vi "VIH - VI Doc Editor - Dialog - Apply Changes.vi"(7 "Title":string, 11 "msg in":string) -> (0 "action":T1(ring))   [LabVIEW 2014]
doc: "::: VI Helpeks :::\nCopyright (c) 2000-2026 Konstantin Shifershteyn. All rights reserved."
panel:
  out "message":string
  in  "SaveVI":bool caption="Save VI after apply"
  in  "%DontApply":bool caption="Don't apply"
  in  "%Apply":bool caption="Apply"
  in  "%Cancel":bool caption="Cancel"
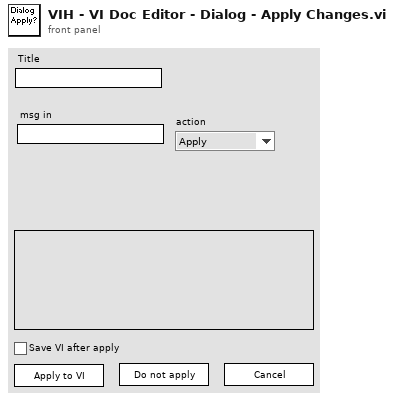
[diagram p1: front panel]
types:
  T1 = enum16{"Apply", "ApplySave", "Continue", "Cancel"}
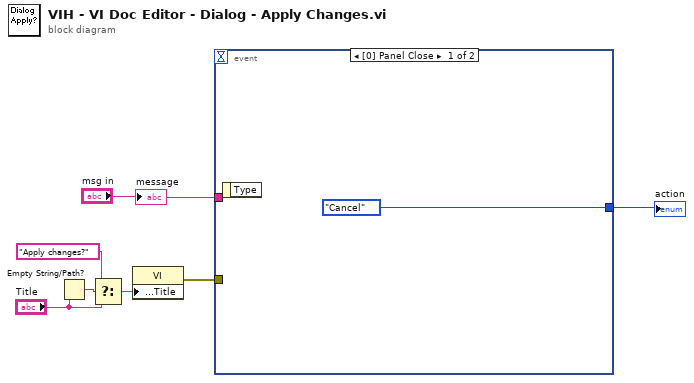
[diagram p0: block diagram]
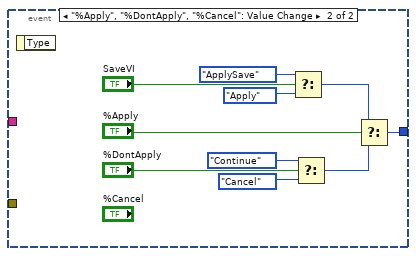
[diagram p2: hidden frame]
diagram:
  n1 = Empty String/Path?(string/path="Title") -> (empty?=w3:bool)
  n2 = Select(t="Apply changes?", s=w3, f="Title") -> (s? t:f=w2:string)
  n3 = property class="VI"("Front Panel.Title"=w2) -> (error out=w5:errorcluster)  [unwired: 2 in, 1 out]
  n4 = event shown="[0] Panel Close" {
    selector: _ -> [_ _]
    dyn-events: _ -> [_ _]
    timeout: _ -> [_ _]
    tunnel: [T1."Cancel" ("action") w18] -> w7
    tunnel: "msg in" -> [_ _]
    tunnel: w5 -> [_ _]
    event Panel Close {
      n5 = event-data() -> ()  [unwired: 1 in, 1 out]
    }
    event "%Apply", "%DontApply", "%Cancel": Value Change {
      n6 = event-data() -> ()  [unwired: 1 in, 1 out]
      n7 = Select(t=T1."ApplySave" ("action"), s="SaveVI", f=T1."Apply" ("action")) -> (s? t:f=w12:T1)
      n8 = Select(t=T1."Continue" ("action"), s="%DontApply", f=T1."Cancel" ("action")) -> (s? t:f=w16:T1)
      n9 = Select(t=w12, s="%Apply", f=w16) -> (s? t:f=w18:T1)
    }
  }
  "action" <- w7
  "message" <- "msg in"
